vi "VIH Project Tree - Find Lost Item Rules.vi"(8 "error in":errorcluster, 11 "Project Tree":T1) -> (0 "error out":errorcluster, 2 "Lost Rules (Owner Paths)":path[](array[path]), 3 "dup Project Tree":T1)   [LabVIEW 2014]
doc: "::: VI Helpeks :::\nCopyright (c) 2000-2026 Konstantin Shifershteyn. All rights reserved."
uses:
  VIH Project Tree Typedef - Tree Refnum.ctl
panel:
  # "VI Helpeks\nCopyright (c) 2012-2026 Konstantin Shifershteyn"
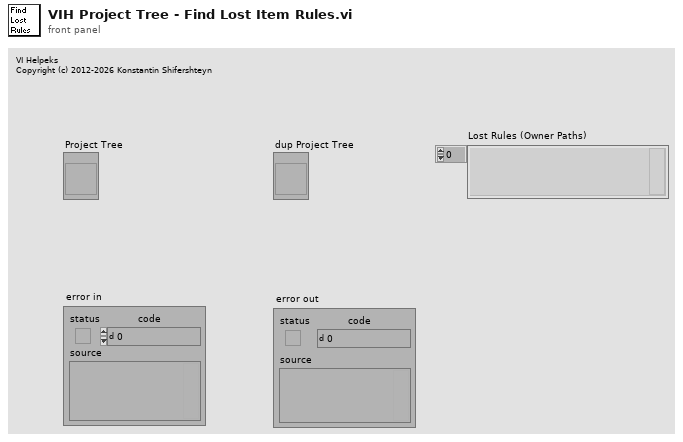
[diagram p1: front panel]
types:
  T1 = typedef "VIH Project Tree Typedef - Tree Refnum.ctl" = refnum<vi>
  T2 = enum16{"get", "get all", "set", "Init", "delete", "rename"}
  T3 = typedef "VIH HelpGen Typedef - Palette - Item Type Enum.ctl" = enum32{"<Invalid>", "<unknown>", "VI", "Menu", "LV Func", "Express VI", "Poly VI", "CTL", "HTML"}
  T4 = cluster{"Types":T3[], "Paths":path[], "Dynamic":enum16{"Dyn", "Stat", "Both"}[], "Can be built":bool[], "DynFileNotFound":bool[]}
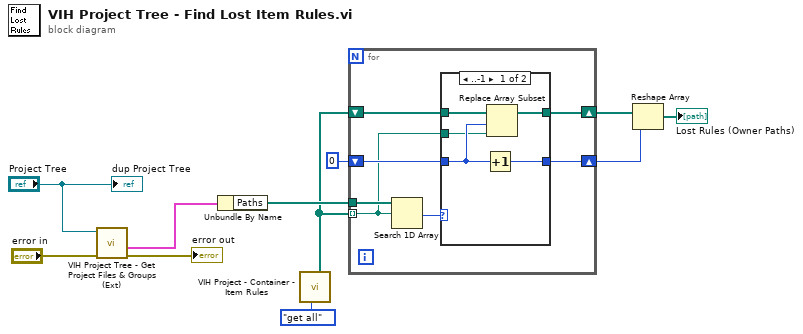
[diagram p0: block diagram]
diagram:
  n1 = call "VIH Project Tree - Get Project Files & Groups (Ext).vi"("error in"="error in", "Project Tree"="Project Tree") -> ("error out"=→"error out":errorcluster, "Project Files"=w1:T4)  [unwired: 6 in, 2 out]
  n2 = Unbundle By Name(w1) -> ("Paths"=w10:path[])
  n3 = call "VIH Project - Container - Item Rules.vi"("cmd (get)"=T2."get all") -> ("Item Paths"=w6:path[])  [unwired: 6 in, 4 out]
  n4 = for {
    tunnel: w10 -> [w18]
    tunnel: w6 -> [w12] mode=indexing
    shift-right: [w14] -> w4
    shift-left: w6 -> [w13]
    shift-right: [w15] -> w3
    shift-left: 0 -> [w16]
    n5 = Search 1D Array(1D array=w18, element=w12) -> (index of element=w17:i32)  [unwired: 1 in]
    n6 = case shown="..-1" w17 {
      tunnel: w16 -> [w21 w25]
      tunnel: [w20 w25] -> w15
      tunnel: [w22 w24] -> w14
      tunnel: w13 -> [w23 w24]
      tunnel: w12 -> [w19 _]
      frame ..-1 {
        n7 = Increment(x=w21) -> (x+1=w20:i32)
        n8 = Replace Array Subset(array=w23, new element=w19, index=w21) -> (w22:path[])
      }
      frame 0.. {
      }
    }
  }
  n9 = Reshape Array(w4, w3) -> (→"Lost Rules (Owner Paths)":path[])
  "dup Project Tree" <- "Project Tree"
